vi "ASD Peak location for Graph VI.vi"(8 "Peak Locations":i32[](array[numeric]) caption="Peak Position", 11 "Region Raw data":dbl[](array[numeric])) -> (3 "Peak Y":dbl[](array[numeric]))   [LabVIEW 2018]
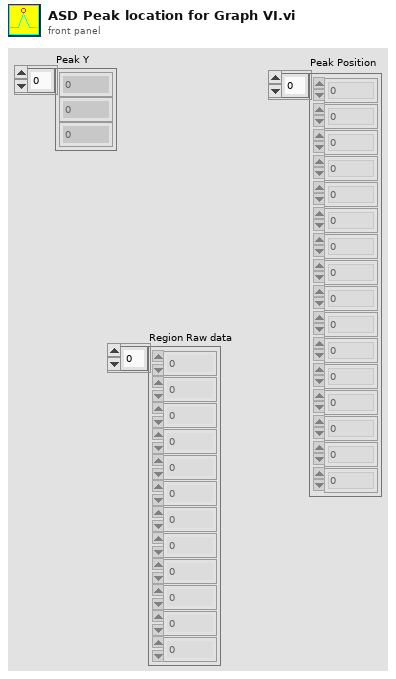
[diagram p1: front panel]
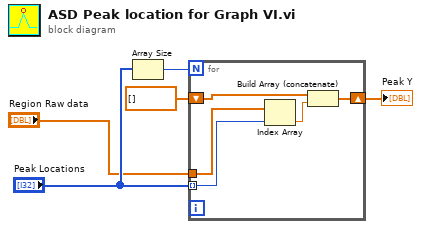
[diagram p0: block diagram]
diagram:
  n1 = Array Size(array="Peak Locations") -> (size(s)=w5:i32)
  n2 = for {
    N: w5 -> [_]
    tunnel: "Peak Locations" -> [w6] mode=indexing
    tunnel: "Region Raw data" -> [w10]
    shift-right: [w9] -> w1
    shift-left: dbl[] [] -> [w8]
    n3 = Index Array(array=w10, index=w6) -> (element=w7:dbl)
    n4 = Build Array (concatenate)(w8, w7) -> (w9:dbl[])
  }
  "Peak Y" <- w1
